vi "Update Task.vi"(7 "Project Store in":refnum<class "Project Store.lvclass">, 8 "error in (no error)":errorcluster, 11 "Task":T1) -> (0 "error out":errorcluster, 3 "found?":bool, 5 "Project Store out":refnum<class "Project Store.lvclass">)   [LabVIEW 2024, in "Project Store.lvclass"]
doc: "Replaces the task whose ID matches the ID in the given row with that row - this is how a rename or a change of the Active flag or Sort Order is made. found? is FALSE and nothing changes when no task has that ID. Nothing is written to disk until Write to Data Source.\n\nGenerated by: Claude"
uses:
  Project Store.lvclass
  Rows/Task.ctl
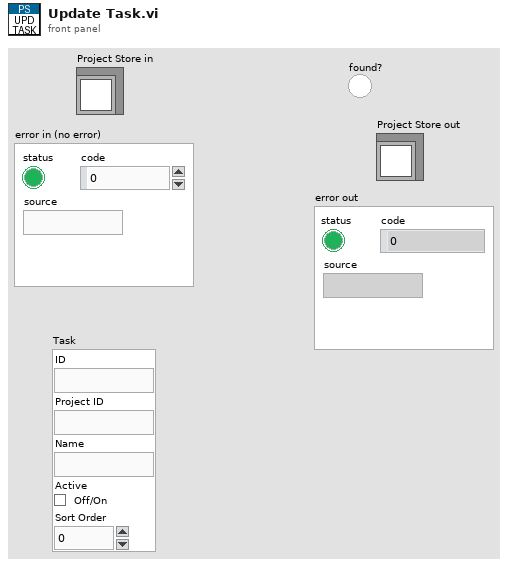
[diagram p1: front panel]
types:
  T1 = typedef "Task.ctl" = cluster{"ID":string, "Project ID":string, "Name":string, "Active":bool, "Sort Order":i32}
  T2 = typedef "Task List.ctl" = T1[]
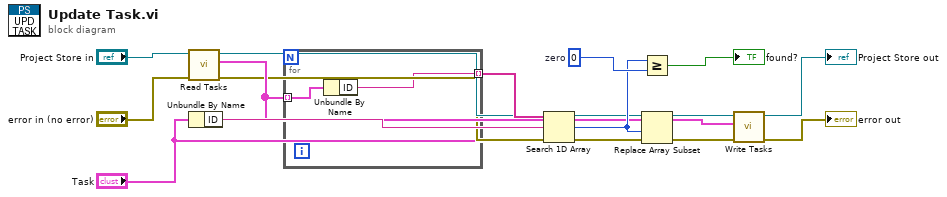
[diagram p0: block diagram]
diagram:
  w10 = 0  # zero
  n1 = call-dynamic "Read Tasks.vi"("error in (no error)"="error in (no error)", "Project Store in"="Project Store in") -> ("error out"=w4:errorcluster, "Task List"=w6:T2, "Project Store out"=w5:refnum<class "Project Store.lvclass">)  [unwired: 7 in]
  n2 = Unbundle By Name("Task") -> ("ID"=w7:string)
  n3 = for {
    tunnel: w6 -> [w15] mode=indexing
    tunnel: [w16] -> w8 mode=indexing
    n4 = Unbundle By Name(w15) -> ("ID"=w16:string)
  }
  n5 = Search 1D Array(1D array=w8, element=w7) -> (index of element=w9:i32)  [unwired: 1 in]
  n6 = Greater Or Equal?(x=w9, y=w10) -> (x >= y?=→"found?":bool)
  n7 = Replace Array Subset(array=w6, new element="Task", index=w9) -> (w12:T2)
  n8 = call-dynamic "Write Tasks.vi"("error in (no error)"=w4, "Task List"=w12, "Project Store in"=w5) -> ("error out"=→"error out":errorcluster, "Project Store out"=→"Project Store out":refnum<class "Project Store.lvclass">)  [unwired: 7 in]
